vi "Condition_Stabilize.vi"(8 "error in (no error)":errorcluster={"status"=FALSE, "code"=0, "source"="\"\""}, 10 "current condition":string, 11 "Previous stable-since":string) -> (0 "error out":errorcluster={"status"=FALSE, "code"=0, "source"="\"\""}, 2 "status ok":bool, 3 "Stable flag and updated timestamp":string)   [LabVIEW 2026]
doc: "INTENT: Require continuous valid completion. LOGIC: Start when TRUE, reset on FALSE/UNKNOWN, report stable only when uninterrupted interval passes."
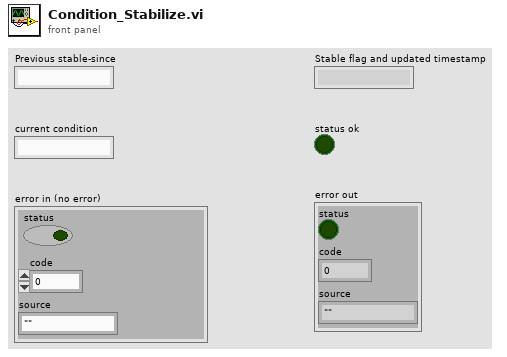
[diagram p1: front panel]
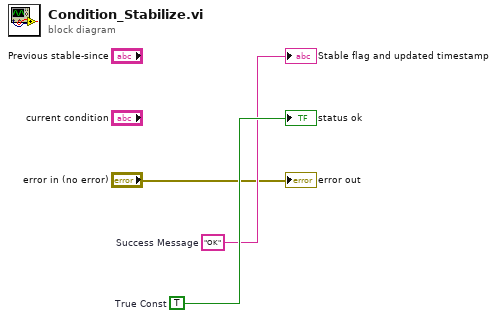
[diagram p0: block diagram]
diagram:
  w3 = TRUE  # True Const
  w2 = "OK"  # Success Message
  "Stable flag and updated timestamp" <- w2
  "status ok" <- w3
  "error out" <- "error in (no error)"
